vi "Sous_VI_Init_machine_etat.vi"(8 "error in (no error)":errorcluster) -> (0 "error out":errorcluster)   [LabVIEW 2017]
uses:
  enum_bras.ctl
  <vilib>/myRIO/Instrument Drivers/Onboard IO/DIO/typedefs/DIO Reference.ctl
  <vilib>/myRIO/Common/Instrument Driver Framework/Utilities/typedefs/myRIO Generic Hardware Reference.ctl
  <vilib>/myRIO/Common/Instrument Driver Framework/Utilities/typedefs/Hardware Version Enum.ctl
  <vilib>/myRIO/Common/Instrument Driver Framework/Utilities/typedefs/myRIO v1.0 Reference.ctl
  <vilib>/myRIO/Common/Instrument Driver Framework/Utilities/typedefs/Generic FPGA Reference.ctl
  <vilib>/myRIO/Common/Instrument Driver Framework/myRIO v1.0/DIO/typedefs/DIO Channels List.ctl
  <vilib>/myRIO/Common/Instrument Driver Framework/myRIO v1.0/DIO/typedefs/DIO Channels Enum.ctl
  <vilib>/userdefined/High Color/nirio_resource_hc.ctl
  <vilib>/myRIO/Common/Instrument Driver Framework/Utilities/vis/Is FPGA Ref Available.vi
  <vilib>/myRIO/Common/Instrument Driver Framework/myRIO v1.0/DIO/vis/myRIO v1.1 Open DIO.vi
  <vilib>/myRIO/Instrument Drivers/Onboard IO/DIO/vis/Write.vi
  <vilib>/myRIO/Instrument Drivers/Onboard IO/DIO/vis/Read.vi
  <vilib>/myRIO/Common/Instrument Driver Framework/Utilities/vis/Validate Channels.vi
  <vilib>/myRIO/Common/Instrument Driver Framework/myRIO v1.0/DIO/vis/myRIO v1.0 Reserve DIO.vi
  <vilib>/myRIO/Common/Instrument Driver Framework/myRIO v1.0/Resource Manager/vis/myRIO v1.0 Reserve Channel List.vi
  <vilib>/myRIO/Common/Instrument Driver Framework/myRIO v1.0/DIO/vis/myRIO v1.0 Build MUX Configuration DIO.vi
  <vilib>/myRIO/Common/Instrument Driver Framework/myRIO v1.0/Resource Manager/vis/myRIO v1.0 Reserve Channel.vi
  <vilib>/myRIO/Common/Instrument Driver Framework/myRIO v1.0/Resource Manager/vis/myRIO v1.0 Unreserve Channel.vi
  <vilib>/myRIO/Common/Instrument Driver Framework/myRIO v1.0/Resource Manager/vis/myRIO v1.0 Create Configuration List.vi
  <vilib>/myRIO/Common/Instrument Driver Framework/myRIO v1.0/Resource Manager/vis/myRIO v1.0 Build Mutex Name.vi
  <vilib>/Utility/VariantDataType/GetNumericInfo.vi
  <vilib>/Utility/error.llb/Error Cluster From Error Code.vi
  <vilib>/myRIO/Common/Instrument Driver Framework/myRIO v1.0/myRIO v1.1 Open.vi
  <vilib>/myRIO/Common/Instrument Driver Framework/Utilities/vis/IO Manager.vi
  <vilib>/myRIO/Common/Instrument Driver Framework/Utilities/vis/Configuration Manager.vi
  <vilib>/myRIO/Common/Instrument Driver Framework/myRIO v1.0/Resource Manager/vis/myRIO v1.0 Configure IO.vi
  <vilib>/myRIO/Common/Instrument Driver Framework/myRIO v1.0/myRIO v1.0 Close.vi
  <vilib>/myRIO/Common/Instrument Driver Framework/myRIO v1.0/DIO/vis/myRIO v1.0 Write DIO.vi
  <vilib>/myRIO/Common/Instrument Driver Framework/myRIO v1.0/DIO/vis/myRIO v1.0 Read DIO.vi
  <vilib>/myRIO/Express VI/Onboard Devices/LED/LED Express VI.xnode
  <vilib>/myRIO/Instrument Drivers/Onboard IO/DIO/vis/myRIO DIO Open.xnode
  <vilib>/myRIO/Express VI/Onboard Devices/Button/Button Express VI.xnode
  <vilib>/myRIO/Instrument Drivers/Onboard IO/DIO/DIO.lvlib
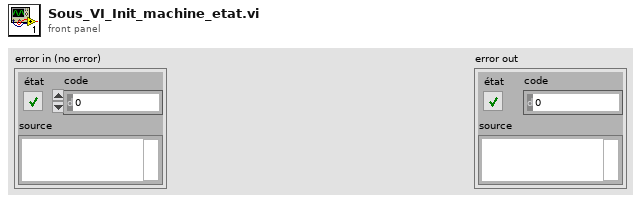
[diagram p1: front panel]
types:
  T1 = typedef "enum_bras.ctl" = enum16{"Depart Bras", "Clapet Bras", "Inactif Bras", "Seaux Bras"}
  T2 = typedef "DIO.lvlib/DIO Reference.ctl" = cluster{"myRIO Reference":T3, "DIO Channels List":T7}
  T3 = typedef "myRIO Generic Hardware Reference.ctl" = cluster{"myRIO Model":T4, "myRIO Hardware Reference":T5}
  T4 = typedef "Hardware Version Enum.ctl" = enum16{"Unknown", "myRIO-1900", "myRIO-1950", "roboRIO", "NI ELVIS RIO CM"}
  T5 = typedef "myRIO v1.0 Reference.ctl" = cluster{"Generic FPGA Reference":T6, "Allow multiple opens":bool}
  T6 = typedef "Generic FPGA Reference.ctl" = refnum<k20>
  T7 = typedef "DIO Channels List.ctl" = T8[]
  T8 = typedef "DIO Channels Enum.ctl" = enum16{"Not Connected", "C/DIO0", "C/DIO1", "C/DIO2", "C/DIO3", "C/DIO4", "C/DIO5", "C/DIO6", "C/DIO7", "A/DIO0", "A/DIO1", "A/DIO2", "A/DIO3", "A/DIO4", "A/DIO5", "A/DIO6", "A/DIO7", "A/DIO8", "A/DIO9", "A/DIO10", "A/DIO11", "A/DIO12", "A/DIO13", "A/DIO14", "A/DIO15", "B/DIO0", "B/DIO1", "B/DIO2", "B/DIO3", "B/DIO4", "B/DIO5", "B/DIO6", "B/DIO7", "B/DIO8", "B/DIO9", "B/DIO10", "B/DIO11", "B/DIO12", "B/DIO13", "B/DIO14", "B/DIO15", "LED0", "LED1", "LED2", "LED3", "Button0", "DIO/DIO0", "DIO/DIO1", "DIO/DIO2", "DIO/DIO3", "DIO/DIO4", "DIO/DIO5", "DIO/DIO6", "DIO/DIO7", "DIO/DIO8", "DIO/DIO9", "SPI/CS0", "SPI/CS1", "SPI/CS2", "SPI/CS3", "LED RADIO (Green)", "LED RADIO (Red)", "LED COMM (Green)", "LED COMM (Red)", "LED MODE (Green)", "LED MODE (Red)"}
  T9 = typedef "nirio_resource_hc.ctl" = tag
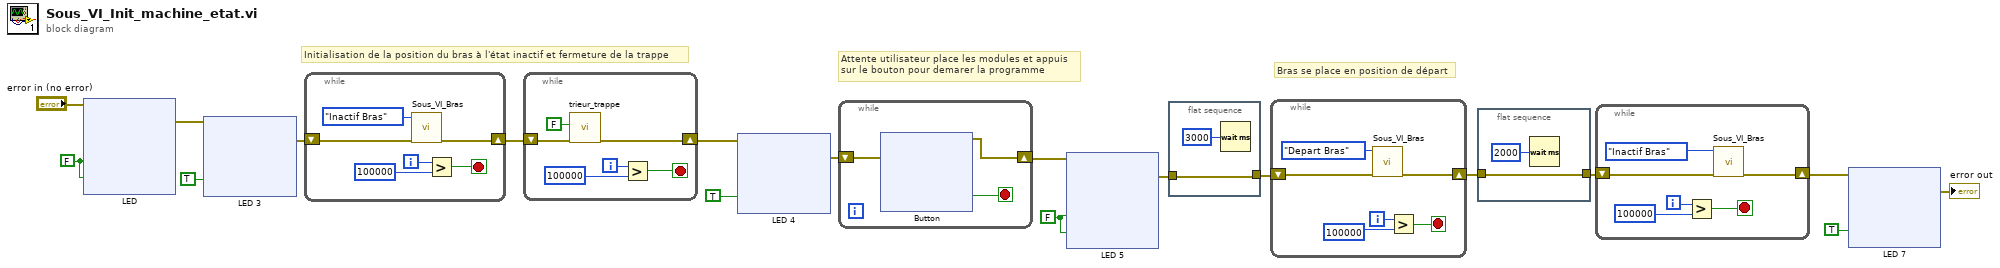
[diagram p0: block diagram]
diagram:
  w5 = FALSE ("LED0")
  w9 = FALSE ("LED0")
  # "Bras se place en position de départ"
  # "Attente utilisateur place les modules et appuis \nsur le bouton pour demarer la programme"
  # "Initialisation de la position du bras à l'état inactif et fermeture de la trappe"
  n1 = xnode "LED"("LED0"=w9, "LED1"=w9, "error in (no error)"="error in (no error)") -> ("error out"=w17:errorcluster)
  n2 = xnode "LED 3"("LED0"=TRUE, "error in (no error)"=w17) -> ("error out"=w7:errorcluster)
  n3 = while {
    shift-right: [w19] -> w16
    shift-left: w7 -> [w20]
    i -> [w23]
    stop <- w21 stop-if-true
    n4 = call "Sous_VI_Bras.vi"("error in (no error)"=w20, "Enum bras"=enum_bras."Inactif Bras") -> ("error out"=w19:errorcluster)  [unwired: 9 in]
    n5 = Greater?(x=w23, y=100000) -> (0:w21:bool)
  }
  n6 = while {
    shift-right: [w25] -> w15
    shift-left: w16 -> [w26]
    i -> [w29]
    stop <- w27 stop-if-true
    n7 = call "trieur_trappe.vi"("error in (no error)"=w26, "Ouvrir"=FALSE) -> ("error out"=w25:errorcluster)  [unwired: 9 in]
    n8 = Greater?(x=w29, y=100000) -> (0:w27:bool)
  }
  n9 = xnode "LED 4"("LED1"=TRUE, "error in (no error)"=w15) -> ("error out"=w14:errorcluster)
  n10 = while {
    shift-right: [w31] -> w13
    shift-left: w14 -> [w32]
    stop <- w33 stop-if-true
    n11 = xnode "Button"("error in (no error)"=w32) -> ("Value"=w33:bool, "error out"=w31:errorcluster)
  }
  n12 = xnode "LED 5"("LED0"=w5, "LED1"=w5, "error in (no error)"=w13) -> ("error out"=w4:errorcluster)
  n13 = flat-sequence {
    tunnel: [w69] -> w12
    tunnel: w4 -> [w69]
    frame #0 {
      n14 = Wait (ms)(milliseconds to wait=u32 3000) -> ()  [unwired: 1 out]
    }
  }
  n15 = while {
    shift-right: [w71] -> w11
    shift-left: w12 -> [w72]
    i -> [w75]
    stop <- w73 stop-if-true
    n16 = call "Sous_VI_Bras.vi"("error in (no error)"=w72, "Enum bras"=enum_bras."Depart Bras") -> ("error out"=w71:errorcluster)  [unwired: 9 in]
    n17 = Greater?(x=w75, y=100000) -> (0:w73:bool)
  }
  n18 = flat-sequence {
    tunnel: [w77] -> w10
    tunnel: w11 -> [w77]
    frame #0 {
      n19 = Wait (ms)(milliseconds to wait=u32 2000) -> ()  [unwired: 1 out]
    }
  }
  n20 = while {
    shift-right: [w79] -> w2
    shift-left: w10 -> [w80]
    i -> [w84]
    stop <- w82 stop-if-true
    n21 = Greater?(x=w84, y=100000) -> (0:w82:bool)
    n22 = call "Sous_VI_Bras.vi"("error in (no error)"=w80, "Enum bras"=enum_bras."Inactif Bras") -> ("error out"=w79:errorcluster)  [unwired: 9 in]
  }
  n23 = xnode "LED 7"("LED1"=TRUE, "error in (no error)"=w2) -> ("error out"=→"error out":errorcluster)
